vi "Remove Inputs with no Paired Output.vi"(8 "error in (no error)":errorcluster, 9 "Paired Module Output Channels":refnum<class "TBM channel.lvclass">[](array[class]), 10 "engine configuration in":refnum<class "engine configuration.lvclass">, 11 "E2E configuration in":refnum<class "E2E Tag Exchange configuration.lvclass">) -> (0 "error out":errorcluster, 2 "engine configuration out":refnum<class "engine configuration.lvclass">, 3 "E2E configuration out":refnum<class "E2E Tag Exchange configuration.lvclass">)   [LabVIEW 2015, in "E2E Tag Exchange editor node.lvclass"]
uses:
  E2E Tag Exchange editor node.lvclass
  <vilib>/NI/Tag Bus Module Framework/channel/TBM channel.lvclass
  <vilib>/NI/Module Execution Interface/Engine Configuration/engine configuration.lvclass
  module/configuration/E2E Tag Exchange configuration.lvclass
  module/configuration/E2E Tag Exchange configuration.lvclass/E2E Tag Exchange configuration.ctl
  <vilib>/NI/Tag Bus Module Framework/channel/channel classification.ctl
  <vilib>/NI/Tag Bus/tag/tag descriptor.lvclass/tag descriptor.ctl
  <vilib>/NI/Tag Bus Module Framework/channel/TBM channel.lvclass/TBM channel.ctl
  <vilib>/NI/Configuration Framework/serializable configuration/NISE_CEF_serializable configuration.lvclass/NISE_CEF_serializable configuration.ctl
  <vilib>/Utility/LVClass/Get LV Class Name.vi
  <vilib>/NI/Configuration Framework/error generator/NISE_error generator.vi
  <vilib>/NI/Configuration Framework/serializable configuration/NISE_CEF_serializable configuration.lvclass
  <vilib>/NI/Tag Bus/tag/tag descriptor.lvclass
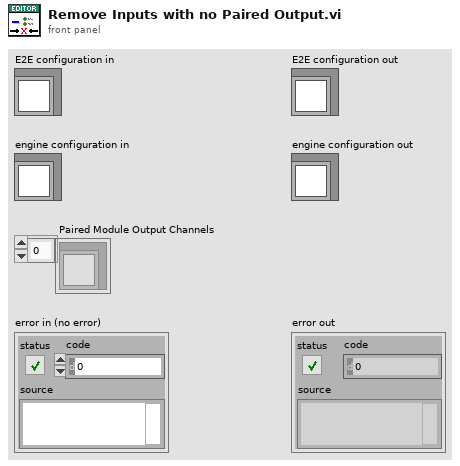
[diagram p1: front panel]
types:
  T1 = typedef "TBM channel.lvclass/channel classification.ctl" = enum16{"input data", "output data", "processing parameter", "processing result"}
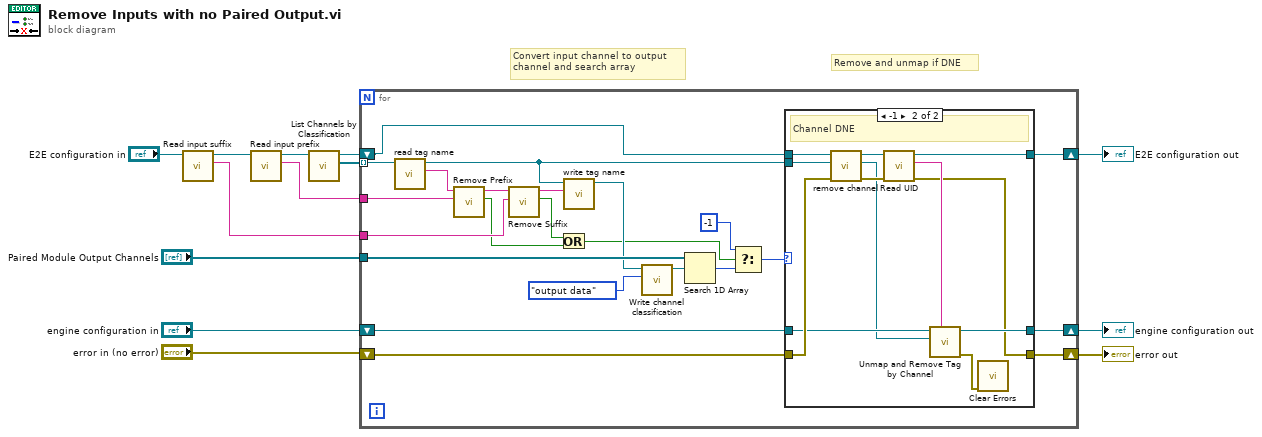
[diagram p0: block diagram]
diagram:
  # "Remove and unmap if DNE"
  # "Convert input channel to output\nchannel and search array"
  n1 = call "Read input suffix.vi"("E2E Tag Exchange configuration in"="E2E configuration in") -> ("input suffix"=w4:string, "E2E Tag Exchange configuration out"=w2:refnum<class "E2E Tag Exchange configuration.lvclass">)  [unwired: 8 in, 1 out]
  n2 = call "Read input prefix.vi"("E2E Tag Exchange configuration in"=w2) -> ("input prefix"=w1:string, "E2E Tag Exchange configuration out"=w3:refnum<class "E2E Tag Exchange configuration.lvclass">)  [unwired: 8 in, 1 out]
  n3 = call "List Channels by Classification.vi"("E2E configuration in"=w3) -> ("Input Channels"=w11:refnum<class "TBM channel.lvclass">[], "E2E configuration out"=w12:refnum<class "E2E Tag Exchange configuration.lvclass">)  [unwired: 8 in, 1 out]
  n4 = for {
    tunnel: "Paired Module Output Channels" -> [w30]
    tunnel: w11 -> [w27] mode=indexing
    shift-right: [w33] -> w7
    shift-left: "engine configuration in" -> [w35]
    shift-right: [w34] -> w6
    shift-left: w12 -> [w22]
    shift-right: [w32] -> w8
    shift-left: "error in (no error)" -> [w31]
    tunnel: w4 -> [w18]
    tunnel: w1 -> [w17]
    n5 = call <vilib>:"read tag name.vi"("system tag in"=w27) -> ("name"=w20:string, "system tag out"=w26:refnum<class "TBM channel.lvclass">)  [unwired: 8 in, 1 out]
    n6 = call "Remove Prefix.vi"("Prefix"=w17, "String"=w20) -> ("Prefix Missing?"=w15:bool, "String out"=w19:string)  [unwired: 8 in]
    n7 = call "Remove Suffix.vi"("Suffix"=w18, "String"=w19) -> ("Suffix Missing?"=w14:bool, "String out"=w21:string)  [unwired: 8 in]
    n8 = Or(x=w14, y=w15) -> (x .or. y?=w16:bool)
    n9 = call <vilib>:"write tag name.vi"("name"=w21, "system tag in"=w26) -> ("system tag out"=w25:refnum<class "TBM channel.lvclass">)  [unwired: 8 in, 1 out]
    n10 = call <vilib>:"Write channel classification.vi"("channel classification"=channel_classification."output data", "channel in"=w25) -> ("channel out"=w29:refnum<class "TBM channel.lvclass">)  [unwired: 8 in, 1 out]
    n11 = Search 1D Array(1D array=w30, element=w29) -> (index of element=w28:i32)  [unwired: 1 in]
    n12 = Select(t=-1, s=w16, f=w28) -> (s? t:f=w24:i32)
    n13 = case shown="-1" w24 {
      tunnel: w22 -> [w38 w51]
      tunnel: w35 -> [w37 w43]
      tunnel: [w38 w47] -> w34
      tunnel: [w37 w45] -> w33
      tunnel: [w39 w42] -> w32
      tunnel: w31 -> [w39 w50]
      tunnel: w26 -> [_ w49]
      frame Default {
        # "Channel Exists"
      }
      frame -1 {
        # "Channel DNE"
        n14 = call "remove channel.vi"("error in (no error)"=w50, "channel"=w49, "E2E configuration in"=w51) -> ("error out"=w46:errorcluster, "removed channel"=w40:refnum<class "TBM channel.lvclass">, "E2E configuration out"=w48:refnum<class "E2E Tag Exchange configuration.lvclass">)  [unwired: 6 in]
        n15 = call <vilib>:"Read UID.vi"("error in"=w46, "configuration in"=w48) -> ("error out"=w42:errorcluster, "instance id"=w44:string, "configuration out"=w47:refnum<class "E2E Tag Exchange configuration.lvclass">)  [unwired: 7 in]
        n16 = call "Unmap and Remove Tag by Channel.vi"("owner ID"=w44, "channel"=w40, "engine configuration in"=w43) -> ("error out"=w41:errorcluster, "engine configuration out"=w45:refnum<class "engine configuration.lvclass">)  [unwired: 7 in]
        n17 = call <vilib>:"Clear Errors.vi"("error in (no error)"=w41) -> ()  [unwired: 5 in, 2 out]
      }
    }
  }
  "E2E configuration out" <- w6
  "engine configuration out" <- w7
  "error out" <- w8
